vi "VIH HelpGen - HTML - Add Generator Info.vi"(10 "Evaluation":bool, 11 "HTML in":string) -> (3 "HTML out":string)   [LabVIEW 2014]
doc: "::: VI Helpeks :::\nCopyright (c) 2000-2026 Konstantin Shifershteyn. All rights reserved."
panel:
  # "VI Helpeks\nCopyright (c) 2012-2026 Konstantin Shifershteyn"
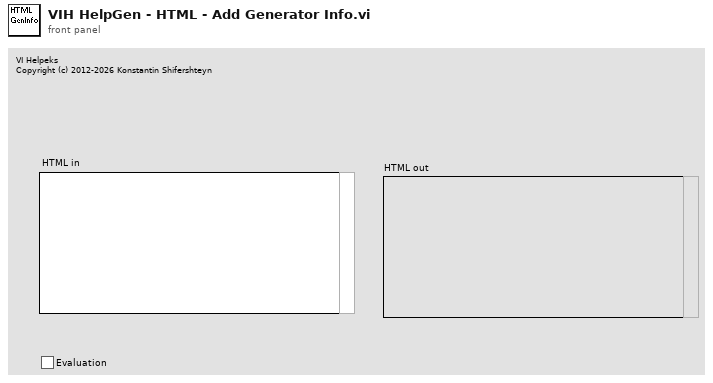
[diagram p1: front panel]
types:
  T1 = cluster{"Product Name":string, "Short Name":string, "Product Version":string, "Release Timestamp":string, "Developer":string, "Copyright":string}
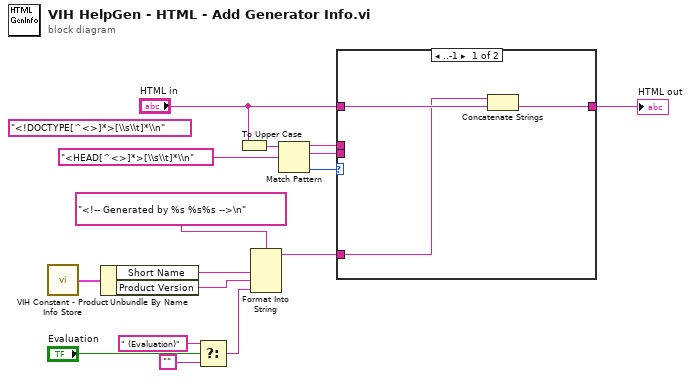
[diagram p0: block diagram]
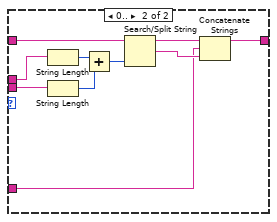
[diagram p2: hidden frame]
diagram:
  (unwired) "<!DOCTYPE[^<>]*>[\\s\\t]*\\n"
  n1 = call "VIH Constant - Product Info Store.vi"() -> ("Product Info"=w16:T1)
  n2 = Unbundle By Name(w16) -> ("Short Name"=w14:string, "Product Version"=w13:string)
  n3 = Select(t=" (Evaluation)", s="Evaluation", f="") -> (s? t:f=w9:string)
  n4 = To Upper Case(1:"HTML in") -> (0:w7:string)
  n5 = Format Into String(format string="<!-- Generated by %s %s%s -->\n", w14, w13, w9) -> (resulting string=w2:string)  [unwired: 2 in, 1 out]
  n6 = Match Pattern(string=w7, regular expression="<HEAD[^<>]*>[\\s\\t]*\\n") -> (before substring=w4:string, match substring=w3:string, offset past match=w6:i32)  [unwired: 1 in, 1 out]
  n7 = case shown="..-1" w6 {
    tunnel: [w18 w21] -> w1
    tunnel: "HTML in" -> [w19 w29]
    tunnel: w4 -> [_ w28]
    tunnel: w3 -> [_ w27]
    tunnel: w2 -> [w17 w20]
    frame ..-1 {
      n8 = Concatenate Strings(w17, w19) -> (w18:string)
    }
    frame 0.. {
      n9 = String Length(string=w28) -> (length=w25:i32)
      n10 = String Length(string=w27) -> (length=w26:i32)
      n11 = Add(x=w25, y=w26) -> (x+y=w24:i32)
      n12 = Search/Split String(string=w29, offset (0)=w24) -> (substring before match=w23:string, match + rest of string=w22:string)  [unwired: 1 in, 1 out]
      n13 = Concatenate Strings(w23, w20, w22) -> (w21:string)
    }
  }
  "HTML out" <- w1
